vi "GV_TC1.vi"() -> ()   [LabVIEW 2025]
panel:
  out "TC1_Command":dbl
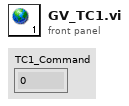
[diagram p1: front panel]
diagram:
